vi "FunctionObjects_Load All.vi"(0 "scripts manager in":refnum<class "scripts manager.lvclass">, 5 "Function Objects In":T1(array[cluster]), 11 "error in (no error)":errorcluster) -> (4 "scripts manager out":refnum<class "scripts manager.lvclass">, 15 "error out":errorcluster)   [LabVIEW 2020, in "LSL.lvlib" / "scripts manager.lvclass"]
uses:
  scripts manager.lvclass
  functions/functionsbase/functionbase.lvclass
  scripts manager.lvclass/scripts manager.ctl
  functions/functionsbase/functionbase.lvclass/functionbase.ctl
  functions/functionsbase/properties/Write Output Terminal.vi
  functions/functionsbase/properties/Write RT Variables.vi
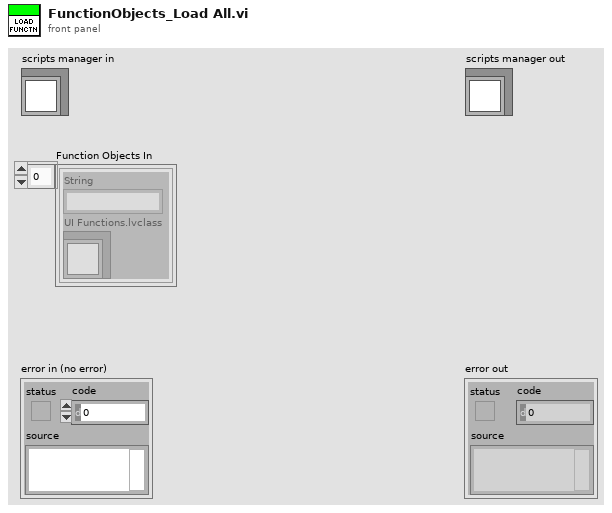
[diagram p1: front panel]
types:
  T1 = cluster{"String":string, "UI Functions.lvclass":refnum<class "functionbase.lvclass">}[]
  T2 = typedef "Scan Syntax Format.ctl" = cluster{"Format String":string, "Variable#":i32, "Variables Name":string[]}
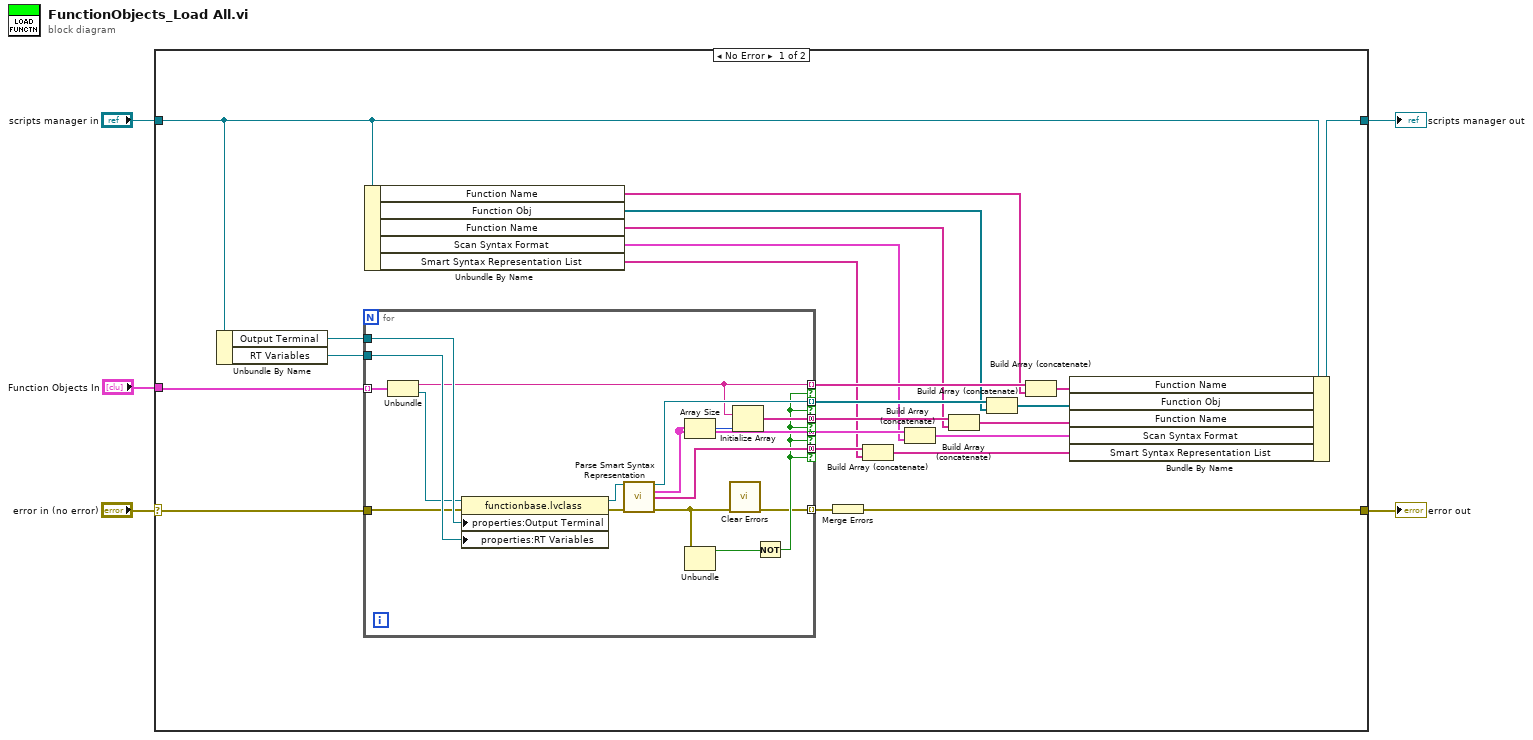
[diagram p0: block diagram]
diagram:
  n1 = case shown="No Error" "error in (no error)" {
    selector: "error in (no error)" -> [w6 w47]
    tunnel: [w23 w47] -> w4
    tunnel: [w24 w46] -> w2
    tunnel: "scripts manager in" -> [w10 w46]
    tunnel: "Function Objects In" -> [w7 _]
    frame No Error {
      n2 = Unbundle By Name(w10) -> ("Output Terminal"=w9:refnum<class "Output Terminal.lvclass">, "RT Variables"=w8:refnum<class "RT Variables.lvclass">)
      n3 = for {
        tunnel: w6 -> [w29]
        tunnel: w7 -> [w32] mode=indexing
        tunnel: [w33] -> w28 mode=indexing
        tunnel: [w43] -> w21 mode=indexing if=w38
        tunnel: [w31] -> w22 mode=indexing if=w38
        tunnel: [w42] -> w27 mode=concatenating if=w38
        tunnel: [w40] -> w25 mode=concatenating if=w38
        tunnel: [w39] -> w26 mode=concatenating if=w38
        tunnel: w9 -> [w35]
        tunnel: w8 -> [w34]
        n4 = Unbundle(w32) -> ("String"=w31:string, "UI Functions.lvclass"=w30:refnum<class "functionbase.lvclass">)
        n5 = property class="functionbase.lvclass"(reference=w30, error in=w29, "properties:Output Terminal"=w35, "properties:RT Variables"=w34) -> (reference out=w36:refnum<class "functionbase.lvclass">, error out=w37:errorcluster)
        n6 = call-dynamic "Parse Smart Syntax Representation.vi"("functionbase in"=w36, "error in (no error)"=w37) -> ("functionbase out"=w43:refnum<class "functionbase.lvclass">, "Scan Syntax List"=w42:T2[], "Smart Syntax Representation List"=w39:string[], "error out"=w44:errorcluster)  [unwired: 10 in]
        n7 = Array Size(array=w42) -> (size(s)=w41:i32)
        n8 = Unbundle(w44) -> ("status"=w45:bool)  [unwired: 2 out]
        n9 = call <vilib>:"Clear Errors.vi"("error in (no error)"=w44) -> ("error out"=w33:errorcluster)  [unwired: 5 in, 1 out]
        n10 = Initialize Array(w31, w41) -> (w40:string[])
        n11 = Not(x=w45) -> (.not. x?=w38:bool)
      }
      n12 = Unbundle By Name(w10) -> ("Function Name"=w19:string[], "Function Obj"=w17:refnum<class "functionbase.lvclass">[], "Function Name"=w15:string[], "Scan Syntax Format"=w13:T2[], "Smart Syntax Representation List"=w11:string[])
      n13 = Merge Errors(w28) -> (w23:errorcluster)
      n14 = Build Array (concatenate)(w26, w11) -> (w12:string[])
      n15 = Build Array (concatenate)(w27, w13) -> (w14:T2[])
      n16 = Build Array (concatenate)(w25, w15) -> (w16:string[])
      n17 = Build Array (concatenate)(w21, w17) -> (w18:refnum<class "functionbase.lvclass">[])
      n18 = Build Array (concatenate)(w22, w19) -> (w20:string[])
      n19 = Bundle By Name(cluster=w10, "Function Name"=w20, "Function Obj"=w18, "Function Name"=w16, "Scan Syntax Format"=w14, "Smart Syntax Representation List"=w12) -> (w24:refnum<class "scripts manager.lvclass">)
    }
    frame Error {
    }
  }
  "error out" <- w4
  "scripts manager out" <- w2
